vi "Ping.vi"(0 "obj in":refnum<class "No Override.lvclass">) -> (1 "obj out":refnum<class "No Override.lvclass">)   [LabVIEW 2026, in "No Override.lvclass"]
doc: "Round14: an ordinary method on a class that implements Can Scale but does NOT override Scale By - the one thing that is supposed to break the whole class. Its existence is what makes the breakage readable: a member to ask the execution state of."
uses:
  No Override.lvclass
  No Override.lvclass/No Override.ctl
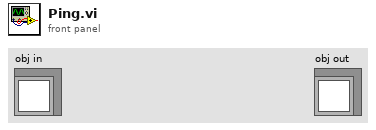
[diagram p1: front panel]
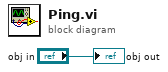
[diagram p0: block diagram]
diagram:
  "obj out" <- "obj in"
